vi "measure BTLE Burst Power.vi"(8 "error in (no error)":errorcluster, 11 "SA Measurement in":refnum<class "SA Measurement.lvclass">) -> (0 "error out":errorcluster, 2 "TXP Value":dbl, 3 "SA Measurement out":refnum<class "SA Measurement.lvclass">)   [LabVIEW 2023, in "Spectrum Analyzer.lvlib" / "SA Measurement.lvclass"]
uses:
  SA Measurement.lvclass
  SA Measurement.lvclass/SA Measurement.ctl
  TYPE DEFINITION/Keysight 9020A/TYPE Measurement Preset.ctl
  Spectrum Analyzer.lvlib
  Interface_Spectrum/Interface_Spectrum.lvclass
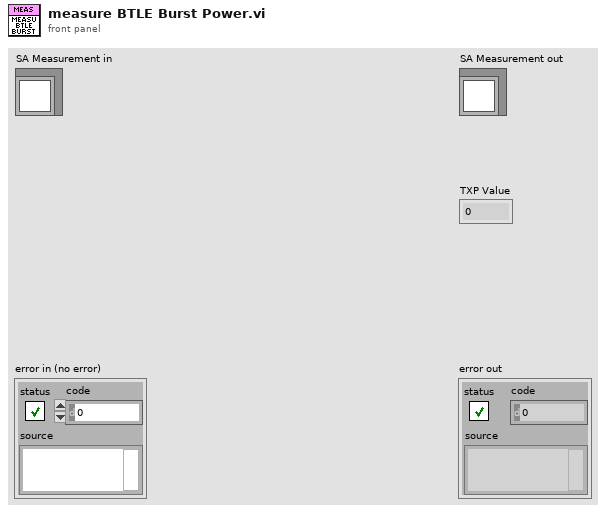
[diagram p1: front panel]
types:
  T1 = typedef "Spectrum Analyzer.lvlib/TYPE Measurement Preset.ctl" = enum16{"Sweep SA Mode", "Channel Power", "Occupied BW", "ACP", "Spurious Emission", "Spurious Emission Mask", "Burst Power (Transmit Power)"}
  T2 = typedef "Spectrum Analyzer.lvlib/TYPE Reference Level and Atten Param.ctl" = cluster{"Reference Level":dbl, "Atten":i32, "Atten Auto?":bool, "Reference Level Offset":dbl}
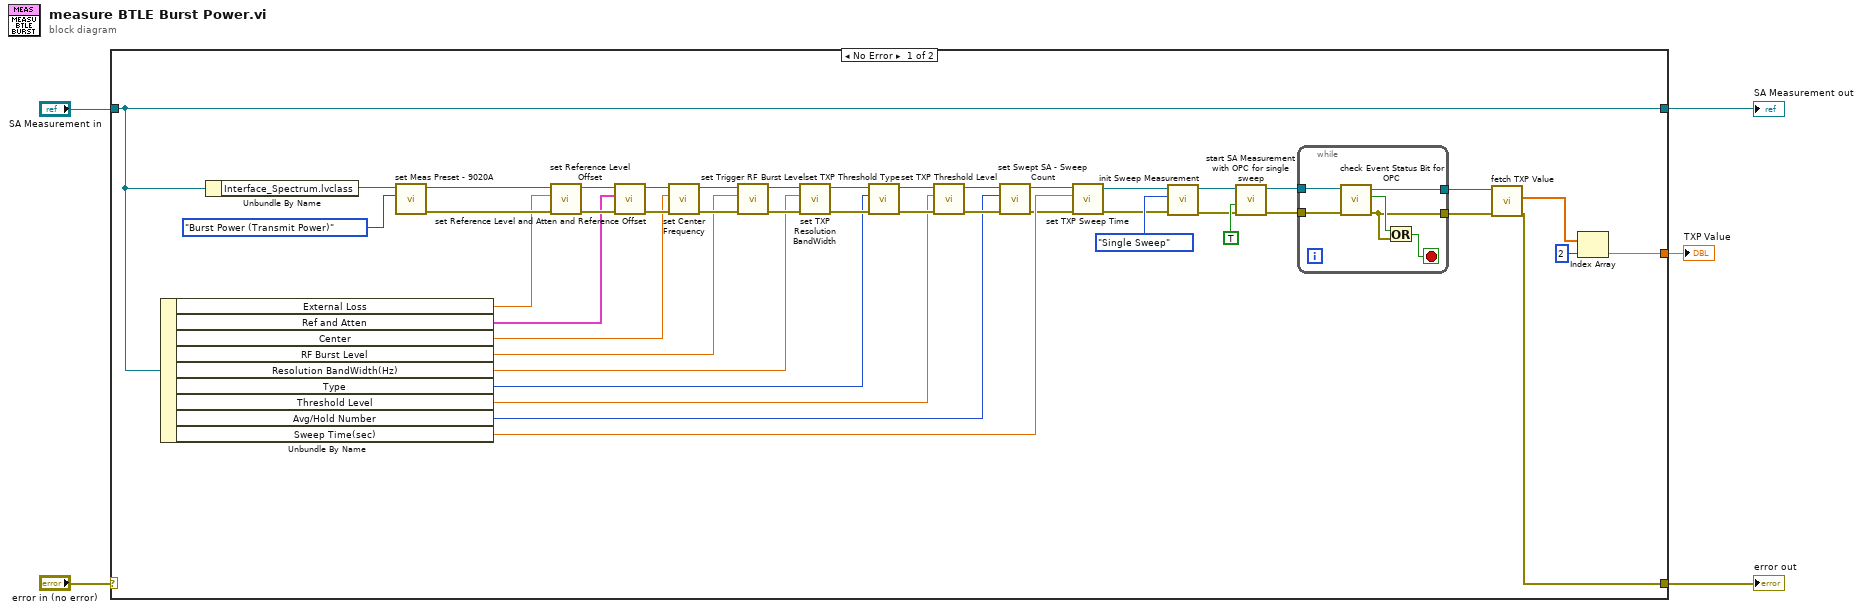
[diagram p0: block diagram]
diagram:
  n1 = case shown="No Error" "error in (no error)" {
    selector: "error in (no error)" -> [_ w57]
    tunnel: [w7 w57] -> w2
    tunnel: [w40 w56] -> w3
    tunnel: "SA Measurement in" -> [w40 w56]
    tunnel: [w6 _] -> w1
    frame No Error {
      n2 = Unbundle By Name(w40) -> ("External Loss"=w43:dbl, "Ref and Atten"=w42:T2, "Center"=w37:dbl, "RF Burst Level"=w29:dbl, "Resolution BandWidth(Hz)"=w26:dbl, "Type"=w23:enum16{"Absolute", "Relative"}, "Threshold Level"=w20:dbl, "Avg/Hold Number"=w17:u32, "Sweep Time(sec)"=w15:dbl)
      n3 = Unbundle By Name(w40) -> ("Interface_Spectrum.lvclass"=w49:refnum<class "Interface_Spectrum.lvclass">)
      n4 = call-dynamic "set Meas Preset - 9020A.vi"("Measurement Preset"=TYPE_Measurement_Preset."Burst Power (Transmit Power)", "Interface_Spectrum in"=w49) -> ("error out"=w46:errorcluster, "Interface_Spectrum out"=w47:refnum<class "Interface_Spectrum.lvclass">)  [unwired: 8 in]
      n5 = call-dynamic "set Reference Level Offset.vi"("error in (no error)"=w46, "Reference Level Offset"=w43, "Interface_Spectrum in"=w47) -> ("error out"=w44:errorcluster, "Interface_Spectrum out"=w45:refnum<class "Interface_Spectrum.lvclass">)  [unwired: 7 in]
      n6 = call-dynamic "set Reference Level and Atten and Reference Offset.vi"("error in (no error)"=w44, "Reference Level, Atten, Reference Offset"=w42, "Interface_Spectrum in"=w45) -> ("error out"=w38:errorcluster, "Interface_Spectrum out"=w39:refnum<class "Interface_Spectrum.lvclass">)  [unwired: 7 in]
      n7 = call-dynamic "set Center Frequency.vi"("error in (no error)"=w38, "Center Frequency (Hz)"=w37, "Interface_Spectrum in"=w39) -> ("error out"=w30:errorcluster, "Interface_Spectrum out"=w31:refnum<class "Interface_Spectrum.lvclass">)  [unwired: 7 in]
      n8 = call-dynamic "set Trigger RF Burst Level.vi"("error in (no error)"=w30, "ABS level (dBm)"=w29, "Interface_Spectrum in"=w31) -> ("error out"=w27:errorcluster, "Interface_Spectrum out"=w28:refnum<class "Interface_Spectrum.lvclass">)  [unwired: 7 in]
      n9 = call-dynamic "set TXP Resolution BandWidth.vi"("error in (no error)"=w27, "BW Value (Hz)"=w26, "Interface_Spectrum in"=w28) -> ("error out"=w24:errorcluster, "Interface_Spectrum out"=w25:refnum<class "Interface_Spectrum.lvclass">)  [unwired: 7 in]
      n10 = call-dynamic "set TXP Threshold Type.vi"("error in (no error)"=w24, "Type"=w23, "Interface_Spectrum in"=w25) -> ("error out"=w21:errorcluster, "Interface_Spectrum out"=w22:refnum<class "Interface_Spectrum.lvclass">)  [unwired: 7 in]
      n11 = call-dynamic "set TXP Threshold Level.vi"("error in (no error)"=w21, "Threshold Level"=w20, "Interface_Spectrum in"=w22) -> ("error out"=w18:errorcluster, "Interface_Spectrum out"=w19:refnum<class "Interface_Spectrum.lvclass">)  [unwired: 7 in]
      n12 = call-dynamic "set Swept SA - Sweep Count.vi"("error in (no error)"=w18, "Sweep Count"=w17, "Interface_Spectrum in"=w19) -> ("error out"=w14:errorcluster, "Interface_Spectrum out"=w16:refnum<class "Interface_Spectrum.lvclass">)  [unwired: 7 in]
      n13 = call-dynamic "set TXP Sweep Time.vi"("error in (no error)"=w14, "Sweep Time(sec)"=w15, "Interface_Spectrum in"=w16) -> ("error out"=w12:errorcluster, "Interface_Spectrum out"=w13:refnum<class "Interface_Spectrum.lvclass">)  [unwired: 7 in]
      n14 = call-dynamic "init Sweep Measurement.vi"("error in (no error)"=w12, "Sweep Measurement Mode"=enum16{"Single Sweep", "Continuous Sweep"}."Single Sweep", "Interface_Spectrum in"=w13) -> ("error out"=w34:errorcluster, "Interface_Spectrum out"=w35:refnum<class "Interface_Spectrum.lvclass">)  [unwired: 7 in]
      n15 = call-dynamic "start SA Measurement with OPC for single sweep.vi"("error in (no error)"=w34, "with OPC?"=TRUE, "Interface_Spectrum in"=w35) -> ("error out"=w32:errorcluster, "Interface_Spectrum out"=w33:refnum<class "Interface_Spectrum.lvclass">)  [unwired: 7 in]
      n16 = while {
        tunnel: w33 -> [w55]
        tunnel: w32 -> [w54]
        tunnel: [w51] -> w10
        tunnel: [w50] -> w11
        stop <- w52 stop-if-true
        n17 = call-dynamic "check Event Status Bit for OPC.vi"("error in (no error)"=w54, "Interface_Spectrum in"=w55) -> ("error out"=w51:errorcluster, "OPC Bit Changed?"=w53:bool, "Interface_Spectrum out"=w50:refnum<class "Interface_Spectrum.lvclass">)  [unwired: 7 in]
        n18 = Or(x=w53, y=w51) -> (x .or. y?=w52:bool)
      }
      n19 = call-dynamic "fetch TXP Value.vi"("error in (no error)"=w10, "Interface_Spectrum in"=w11) -> ("error out"=w7:errorcluster, "TXP Value"=w8:dbl[])  [unwired: 7 in, 1 out]
      n20 = Index Array(array=w8, index=2) -> (element=w6:dbl)
    }
    frame Error {
    }
  }
  "error out" <- w2
  "SA Measurement out" <- w3
  "TXP Value" <- w1
